vi "OPC Client.vi"(0 "Sequence Context In":refnum<k7>, 1 "Operations":T3(ring), 2 "Read":T2={"Value to Read"=enum."Flow Rate", "Timeout"=1.0}, 3 "Read Until":T1={"Timeout"=20.0, "Command"="FLOWRATE", "Measurement Interval"=1.0, "Lo Range Limit"=8.0, "Hi Range Limit"=4.0, "Delta Limit"=0.25, "Default Value"=0.0, "Value Done"=0.0, "Delta Value"=0.0, "Delta Time"=0.0}, 5 "error in":errorcluster, 8 "Comm":cluster{"Station":string, "Process name":string}={"Station"="OP30_1", "Process name"="RTheta"}, 9 "Time Out":cluster{"Continue Testing":bool, "Timeout":dbl}={"Continue Testing"=TRUE, "Timeout"=-1.0}) -> (13 "Fixture No.":string, 14 "comm ok?":bool, 15 "Code":string, 16 "Read Value":string, 17 "Read Until Value":dbl, 19 "error out":errorcluster)   [LabVIEW 2013]
uses:
  read_bool.vi
  read_String.vi
  <vilib>/addons/TestStand/_TSUtility.llb/TestStand - Get Property Value (Boolean).vi
  write_bool.vi
  read_Float.vi
  read_Num.vi
  write_Num.vi
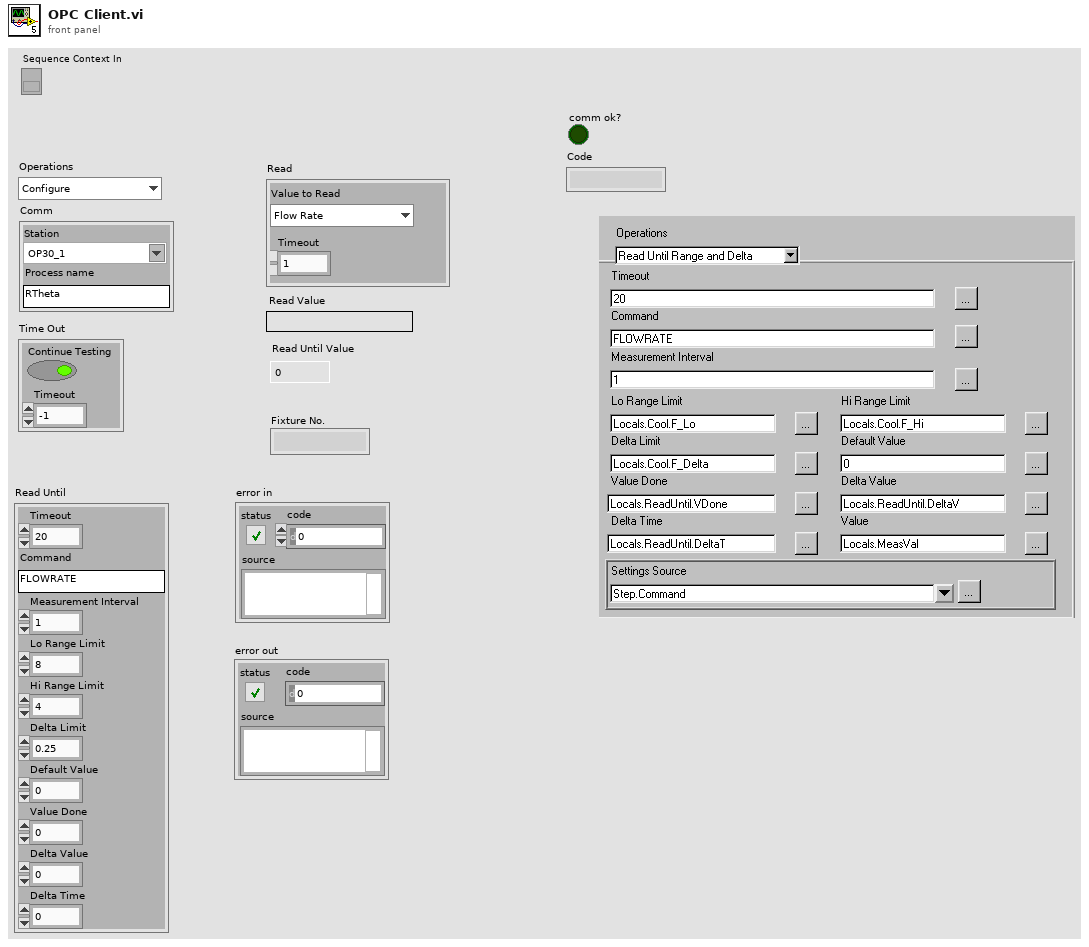
[diagram p1: front panel]
types:
  T1 = cluster{"Timeout":dbl, "Command":string, "Measurement Interval":dbl, "Lo Range Limit":dbl, "Hi Range Limit":dbl, "Delta Limit":dbl, "Default Value":dbl, "Value Done":dbl, "Delta Value":dbl, "Delta Time":dbl}
  T2 = cluster{"Value to Read":enum16{"Flow Rate", "Fluid Temp", "Fluid Fault State", "Temp Fault State", "Coolant Panel State", "Purge Complete", "Seal Test Complete", "Pressure"}, "Timeout":dbl}
  T3 = enum16{"Configure", "Process Name", "Wait Start Test", "Cool", "Read", "Read Until Range and Dellta", "Purge", "Pass", "Fail", "Retry", "Seal Test", "Close"}
  T4 = enum16{"Flow Rate", "Fluid Temp", "Fluid Fault State", "Temp Fault State", "Coolant Panel State", "Purge Complete", "Seal Test Complete", "Pressure"}
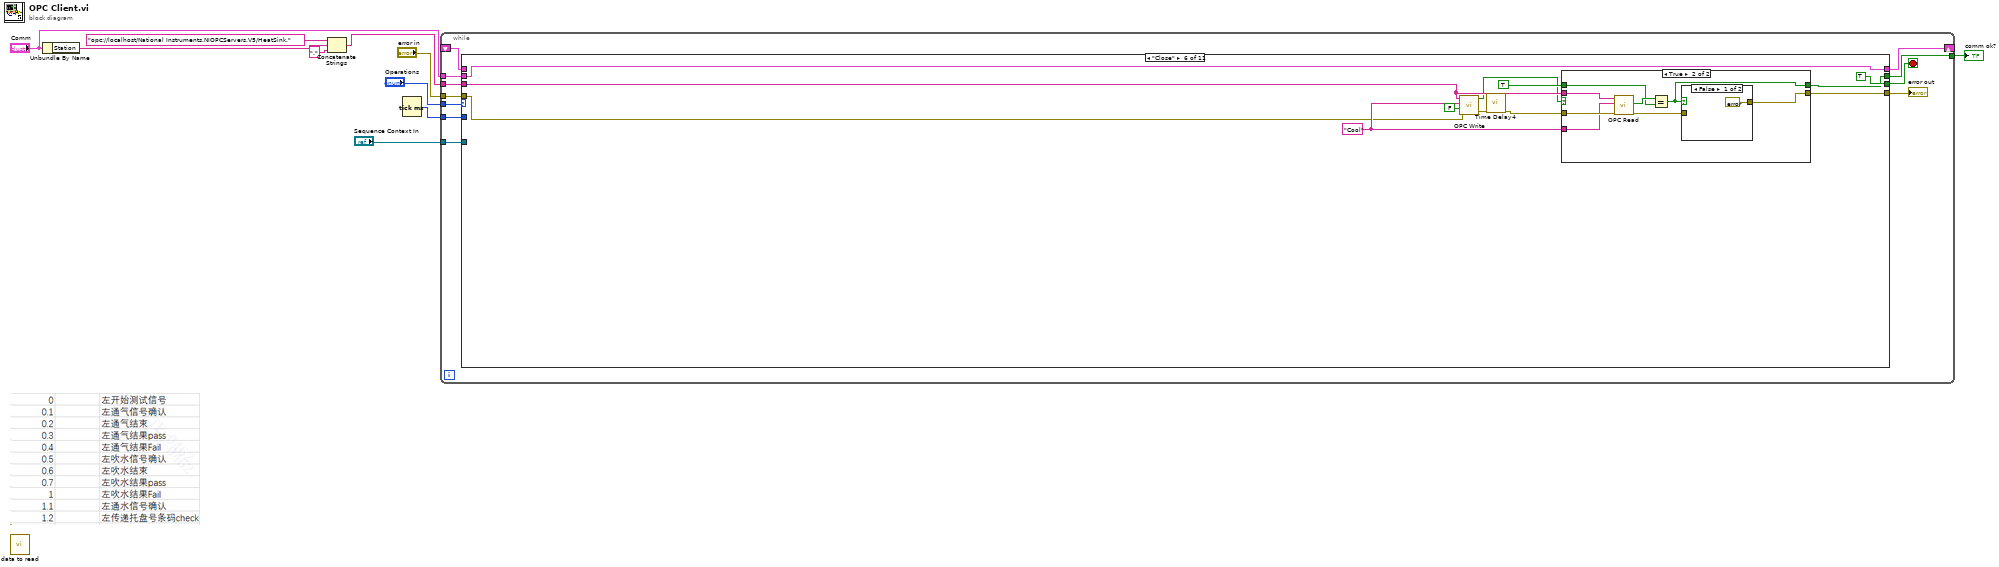
[diagram p0: block diagram]
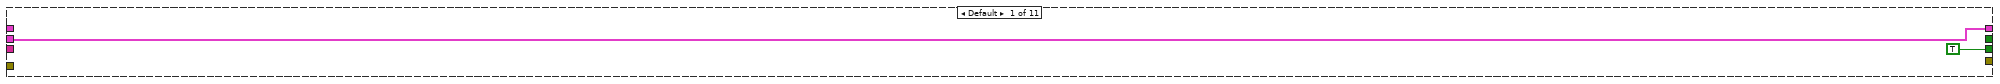
[diagram p2: hidden frame]
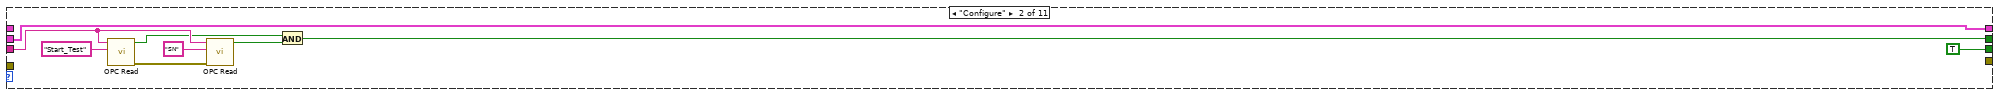
[diagram p3: hidden frame]
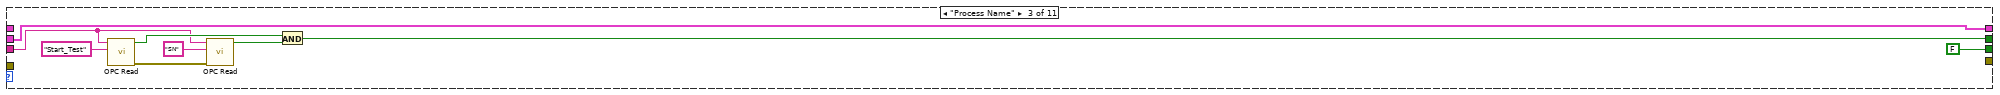
[diagram p4: hidden frame]
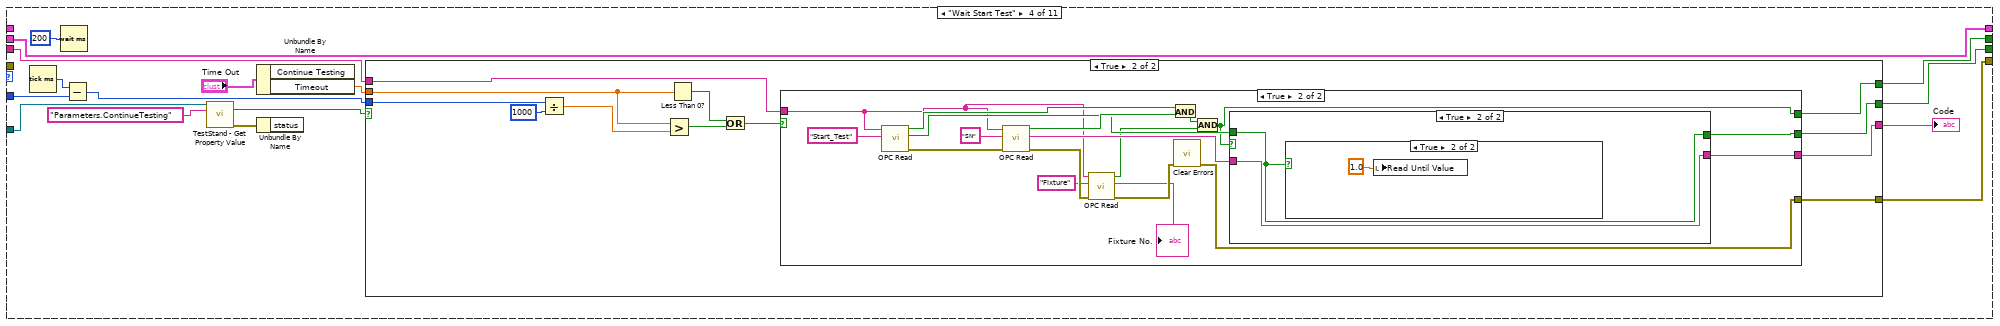
[diagram p5: hidden frame]
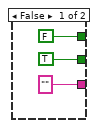
[diagram p6: hidden frame]
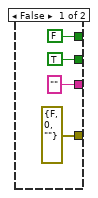
[diagram p7: hidden frame]
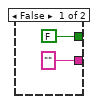
[diagram p8: hidden frame]
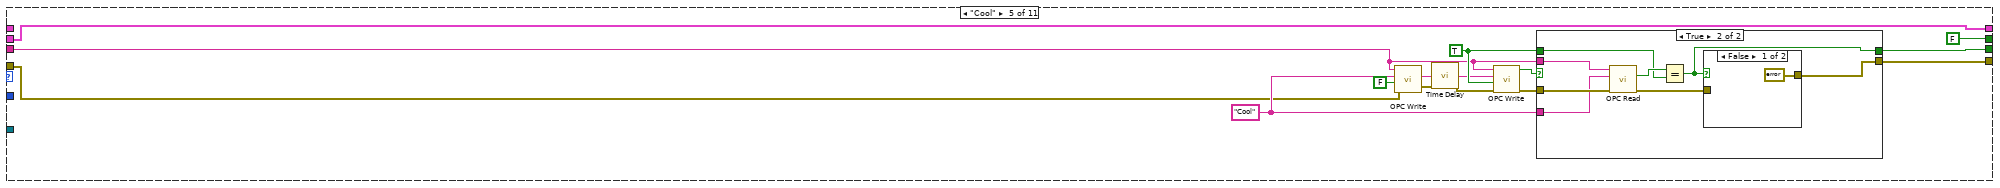
[diagram p10: hidden frame]
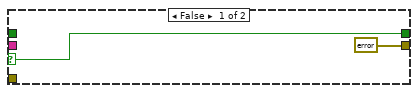
[diagram p11: hidden frame]
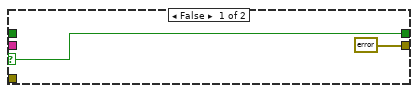
[diagram p13: hidden frame]
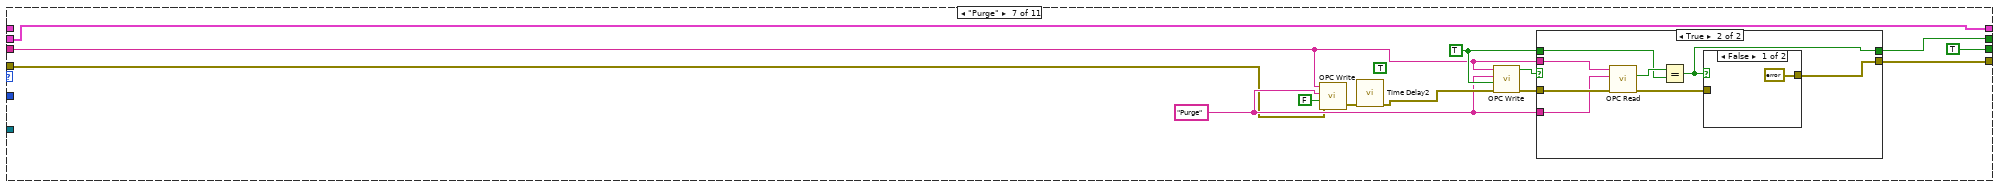
[diagram p15: hidden frame]
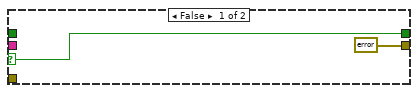
[diagram p16: hidden frame]
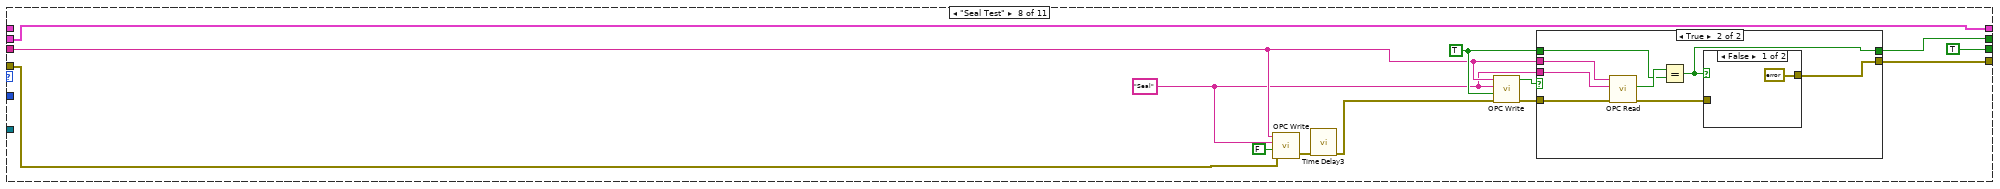
[diagram p18: hidden frame]
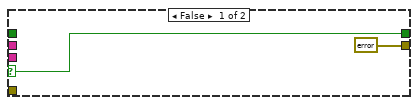
[diagram p19: hidden frame]
diagram:
  n1 = call "data to read.vi"() -> ()  [unwired: 9 in, 3 out]
  n2 = Unbundle By Name("Comm") -> ("Station"=w5:string)
  n3 = Concatenate Strings("opc://localhost/National Instruments.NIOPCServers.V5/HeatSink." ("URL"), w5, "." ("string")) -> (w8:string)
  n4 = Tick Count (ms)() -> (millisecond timer value=w3:u32)
  n5 = while {
    tunnel: w8 -> [w21]
    tunnel: "Operations" -> [w20]
    tunnel: "error in" -> [w19]
    shift-right: [w16] -> _
    shift-left: _ -> [w17]
    tunnel: "Comm" -> [w15]
    tunnel: w3 -> [w12]
    tunnel: "Sequence Context In" -> [w14]
    tunnel: [w11] -> w1
    stop <- w13 stop-if-true
    n6 = case shown="\"Close\"" w20 {
      selector: w20 -> [_ _ _ _ _ _ _ _ _ _ w421]
      tunnel: w21 -> [_ w28 w35 w55 w104 w132 w150 w176 w203 w350 w424]
      tunnel: [_ _ _ w54 w106 w134 w156 w184 w209 w341 w423] -> w18
      tunnel: w19 -> [_ _ _ _ w101 w129 w149 w177 w202 w342 w427]
      tunnel: w17 -> [_ _ _ _ _ _ _ _ _ _ _]
      tunnel: [w23 w32 w41 w57 w112 w136 w161 w183 w208 w353 w422] -> w16
      tunnel: w15 -> [w23 w32 w41 w57 w112 w136 w161 w183 w208 w353 w422]
      tunnel: w14 -> [_ _ _ w46 _ _ _ _ _ _ _]
      tunnel: [TRUE ("Value") TRUE ("Value") FALSE ("Value") w53 w107 TRUE TRUE ("Value") TRUE ("Value") TRUE ("Value") TRUE ("Value") TRUE ("Value")] -> w13
      tunnel: w12 -> [_ _ _ w49 _ _ _ _ _ _ _]
      tunnel: [_ w25 w34 w47 FALSE w125 w157 w181 w199 _ w418] -> w11
      frame Default {
      }
      frame "Configure" {
        n7 = call-poly "OPC Read.vi"("Address"="Start_Test", "URL"=w28) -> ("error out"=w29:errorcluster, "ok?"=w27:bool)  [unwired: 7 in, 1 out]
        n8 = call-poly "OPC Read.vi"("错误输入（无错误）"=w29, "Address"="SN", "URL"=w28) -> ("ok?"=w26:bool)  [unwired: 6 in, 2 out]
        n9 = And(x=w27, y=w26) -> (x .and. y?=w25:bool)
      }
      frame "Process Name" {
        n10 = call-poly "OPC Read.vi"("Address"="Start_Test", "URL"=w35) -> ("error out"=w38:errorcluster, "ok?"=w37:bool)  [unwired: 7 in, 1 out]
        n11 = call-poly "OPC Read.vi"("错误输入（无错误）"=w38, "Address"="SN", "URL"=w35) -> ("ok?"=w36:bool)  [unwired: 6 in, 2 out]
        n12 = And(x=w37, y=w36) -> (x .and. y?=w34:bool)
      }
      frame "Wait Start Test" {
        n13 = Tick Count (ms)() -> (millisecond timer value=w50:u32)
        n14 = Wait (ms)(milliseconds to wait=u32 200) -> ()  [unwired: 1 out]
        n15 = Subtract(x=w50, y=w49) -> (x-y=w48:u32)
        n16 = call-poly <vilib>:"TestStand - Get Property Value.vi"("Sequence Context In"=w46, "Lookup String"="Parameters.ContinueTesting") -> ("Value"=w44:bool, "error out"=w43:errorcluster)  [unwired: 11 in, 1 out]
        n17 = Unbundle By Name("Time Out") -> ("Timeout"=w51:dbl)  [unwired: 1 out]
        n18 = Unbundle By Name(w43) -> ()  [unwired: 1 out]
        n19 = case shown="True" w44 {
          tunnel: w55 -> [_ w72]
          tunnel: [_ w71] -> w54
          tunnel: [TRUE ("Value") w70] -> w53
          tunnel: ["" ("Value") w69] -> w52
          tunnel: w51 -> [_ w63]
          tunnel: w48 -> [_ w66]
          tunnel: [FALSE w61] -> w47
          frame False {
          }
          frame True {
            n20 = Divide(x=w66, y=u32 1000) -> (x/y=w64:dbl)
            n21 = Greater?(x=w63, y=w64) -> (0:w62:bool)
            n22 = Less Than 0?(x=w63) -> (x < 0?=w67:bool)
            n23 = Or(x=w67, y=w62) -> (x .or. y?=w68:bool)
            n24 = case shown="True" w68 {
              tunnel: w72 -> [_ w84]
              tunnel: [errorcluster {"status"=FALSE, "code"=0, "source"=""} ("error out") w91] -> w71
              tunnel: [TRUE ("Value") w87] -> w70
              tunnel: ["" ("Value") w85] -> w69
              tunnel: [FALSE w78] -> w61
              frame False {
              }
              frame True {
                n25 = call-poly "OPC Read.vi"("Address"="Start_Test", "URL"=w84) -> ("error out"=w92:errorcluster, "Value"=w88:bool, "ok?"=w90:bool)  [unwired: 7 in]
                n26 = call-poly "OPC Read.vi"("错误输入（无错误）"=w92, "Address"="SN", "URL"=w84) -> ("error out"=w83:errorcluster, "Value"=w86:string, "ok?"=w89:bool)  [unwired: 6 in]
                n27 = call-poly "OPC Read.vi"("错误输入（无错误）"=w83, "Address"="Fixture", "URL"=w84) -> ("error out"=w82:errorcluster, "Value"=→"Fixture No.":string, "ok?"=w79:bool)  [unwired: 6 in]
                n28 = And(x=w90, y=w89) -> (x .and. y?=w80:bool)
                n29 = call <vilib>:"Clear Errors.vi"("error in (no error)"=w82) -> ("error out"=w91:errorcluster)  [unwired: 6 in]
                n30 = And(x=w80, y=w79) -> (x .and. y?=w78:bool)
                n31 = case shown="True" w78 {
                  tunnel: w88 -> [_ w97]
                  tunnel: [FALSE ("Value") w97] -> w87
                  tunnel: w86 -> [_ w98]
                  tunnel: ["" ("Value") w98] -> w85
                  frame False {
                  }
                  frame True {
                    n32 = case shown="True" w97 {
                      frame False {
                      }
                      frame True {
                        n33 = local write "Read Until Value"(1.0 ("Read Until Value")) -> ()
                      }
                    }
                  }
                }
              }
            }
          }
        }
        "Code" <- w52
      }
      frame "Cool" {
        w108 = TRUE ("Value")
        w105 = "Cool" ("Address")
        n34 = call-poly "OPC Write.vi"("错误输入（无错误）"=w101, "Value"=FALSE, "Address"=w105, "URL"=w104) -> ("error out"=w102:errorcluster)  [unwired: 6 in, 1 out]
        n35 = call "Time Delay"("error in (no error)"=w102) -> ("error out"=w100:errorcluster)  [unwired: 10 in]
        n36 = call-poly "OPC Write.vi"("错误输入（无错误）"=w100, "Value"=w108, "Address"=w105, "URL"=w104) -> ("error out"=w109:errorcluster, "ok?"=w110:bool)  [unwired: 6 in]
        n37 = case shown="True" w110 {
          selector: w110 -> [w113 _]
          tunnel: w109 -> [_ w122]
          tunnel: w104 -> [_ w121]
          tunnel: [errorcluster {"status"=FALSE, "code"=10001, "source"="Write Error"} ("error out") w120] -> w106
          tunnel: [w113 w115] -> w107
          tunnel: w105 -> [_ w118]
          tunnel: w108 -> [_ w116]
          frame False {
          }
          frame True {
            n38 = call-poly "OPC Read.vi"("错误输入（无错误）"=w122, "Address"=w118, "URL"=w121) -> ("error out"=w119:errorcluster, "Value"=w117:bool)  [unwired: 6 in, 1 out]
            n39 = Equal?(x=w117, y=w116) -> (x = y?=w115:bool)
            n40 = case shown="False" w115 {
              tunnel: [errorcluster {"status"=FALSE, "code"=10001, "source"="Check Error"} ("error out") w124] -> w120
              tunnel: w119 -> [_ w124]
              frame False {
              }
              frame True {
              }
            }
          }
        }
      }
      frame "Close" {
        w133 = "Cool" ("Address")
        n41 = call-poly "OPC Write.vi"("错误输入（无错误）"=w129, "Value"=FALSE, "Address"=w133, "URL"=w132) -> ("error out"=w130:errorcluster, "ok?"=w127:bool)  [unwired: 6 in]
        n42 = call "Time Delay4"("error in (no error)"=w130) -> ("error out"=w128:errorcluster)  [unwired: 10 in]
        n43 = case shown="True" w127 {
          selector: w127 -> [w137 _]
          tunnel: w128 -> [_ w146]
          tunnel: w132 -> [_ w145]
          tunnel: [errorcluster {"status"=FALSE, "code"=10001, "source"="Write Error"} ("error out") w144] -> w134
          tunnel: [w137 w139] -> w125
          tunnel: w133 -> [_ w142]
          tunnel: TRUE ("Value") -> [_ w140]
          frame False {
          }
          frame True {
            n44 = call-poly "OPC Read.vi"("错误输入（无错误）"=w146, "Address"=w142, "URL"=w145) -> ("error out"=w143:errorcluster, "Value"=w141:bool)  [unwired: 6 in, 1 out]
            n45 = Equal?(x=w141, y=w140) -> (x = y?=w139:bool)
            n46 = case shown="False" w139 {
              tunnel: [errorcluster {"status"=FALSE, "code"=10001, "source"="Check Error"} ("error out") w148] -> w144
              tunnel: w143 -> [_ w148]
              frame False {
              }
              frame True {
              }
            }
          }
        }
      }
      frame "Purge" {
        (unwired) TRUE ("Value")
        w158 = TRUE ("Value")
        w151 = "Purge" ("Address")
        n47 = call-poly "OPC Write.vi"("错误输入（无错误）"=w149, "Value"=FALSE, "Address"=w151, "URL"=w150) -> ("error out"=w153:errorcluster)  [unwired: 6 in, 1 out]
        n48 = call "Time Delay2"("error in (no error)"=w153) -> ("error out"=w152:errorcluster)  [unwired: 10 in]
        n49 = call-poly "OPC Write.vi"("错误输入（无错误）"=w152, "Value"=w158, "Address"=w151, "URL"=w150) -> ("error out"=w159:errorcluster, "ok?"=w160:bool)  [unwired: 6 in]
        n50 = case shown="True" w160 {
          selector: w160 -> [w162 _]
          tunnel: w159 -> [_ w171]
          tunnel: w150 -> [_ w170]
          tunnel: [errorcluster {"status"=FALSE, "code"=10001, "source"="Write Error"} ("error out") w169] -> w156
          tunnel: [w162 w164] -> w157
          tunnel: w151 -> [_ w167]
          tunnel: w158 -> [_ w165]
          frame False {
          }
          frame True {
            n51 = call-poly "OPC Read.vi"("错误输入（无错误）"=w171, "Address"=w167, "URL"=w170) -> ("error out"=w168:errorcluster, "Value"=w166:bool)  [unwired: 6 in, 1 out]
            n52 = Equal?(x=w166, y=w165) -> (x = y?=w164:bool)
            n53 = case shown="False" w164 {
              tunnel: [errorcluster {"status"=FALSE, "code"=10001, "source"="Check Error"} ("error out") w173] -> w169
              tunnel: w168 -> [_ w173]
              frame False {
              }
              frame True {
              }
            }
          }
        }
      }
      frame "Seal Test" {
        w182 = TRUE ("Value")
        w175 = "Seal" ("Address")
        n54 = call-poly "OPC Write.vi"("错误输入（无错误）"=w177, "Value"=FALSE, "Address"=w175, "URL"=w176) -> ("error out"=w178:errorcluster)  [unwired: 6 in, 1 out]
        n55 = call "Time Delay3"("error in (no error)"=w178) -> ("error out"=w174:errorcluster)  [unwired: 10 in]
        n56 = call-poly "OPC Write.vi"("错误输入（无错误）"=w174, "Value"=w182, "Address"=w175, "URL"=w176) -> ("error out"=w185:errorcluster, "ok?"=w186:bool)  [unwired: 6 in]
        n57 = case shown="True" w186 {
          selector: w186 -> [w187 _]
          tunnel: w185 -> [_ w196]
          tunnel: w176 -> [_ w195]
          tunnel: [errorcluster {"status"=FALSE, "code"=10001, "source"="Write Error"} ("error out") w194] -> w184
          tunnel: [w187 w189] -> w181
          tunnel: w175 -> [_ w192]
          tunnel: w182 -> [_ w190]
          frame False {
          }
          frame True {
            n58 = call-poly "OPC Read.vi"("错误输入（无错误）"=w196, "Address"=w192, "URL"=w195) -> ("error out"=w193:errorcluster, "Value"=w191:bool)  [unwired: 6 in, 1 out]
            n59 = Equal?(x=w191, y=w190) -> (x = y?=w189:bool)
            n60 = case shown="False" w189 {
              tunnel: [errorcluster {"status"=FALSE, "code"=10001, "source"="Check Error"} ("error out") w198] -> w194
              tunnel: w193 -> [_ w198]
              frame False {
              }
              frame True {
              }
            }
          }
        }
      }
      frame "Read" {
        # "1.3-1.6      Seal Cool Purge Bypass\n\n4.3-4.6      Seal Cool Purge Bypass"
        n61 = Unbundle By Name("Read") -> ("Value to Read"=w205:T4)  [unwired: 1 out]
        n62 = case shown="\"Temp Fault State\"" w205 {
          tunnel: ["None" ("Read Value") w215 w225 w242 w269 w281 w299 w312 w331] -> w204
          tunnel: w203 -> [_ w220 w223 w235 w260 w285 w298 w315 w332]
          tunnel: w202 -> [w211 w219 w226 w247 w268 w284 w297 w314 w329]
          tunnel: [w211 w218 w222 w239 w261 w283 w296 w313 w328] -> w201
          tunnel: [TRUE ("ok?") w213 w221 w236 w258 w279 w295 w311 w327] -> w199
          frame Default {
          }
          frame "Flow Rate" {
            n63 = call-poly "OPC Read.vi"("错误输入（无错误）"=w219, "Address"="FlowRate", "URL"=w220) -> ("error out"=w218:errorcluster, "Value"=w214:dbl, "ok?"=w213:bool)  [unwired: 6 in]
            n64 = local write "Read Until Value"(w214) -> ()
            n65 = Format Into String(initial string="%.3f", w214) -> (resulting string=w215:string)  [unwired: 2 in, 1 out]
          }
          frame "Fluid Temp" {
            n66 = call-poly "OPC Read.vi"("错误输入（无错误）"=w226, "Address"="FluidTemp", "URL"=w223) -> ("error out"=w222:errorcluster, "Value"=w224:dbl, "ok?"=w221:bool)  [unwired: 6 in]
            n67 = local write "Read Until Value"(w224) -> ()
            n68 = Format Into String(initial string="%.3f", w224) -> (resulting string=w225:string)  [unwired: 2 in, 1 out]
          }
          frame "Fluid Fault State" {
            n69 = call-poly "OPC Read.vi"("错误输入（无错误）"=w247, "Address"="CoolantState", "URL"=w235) -> ("error out"=w240:errorcluster, "Value"=w246:i32, "ok?"=w237:bool)  [unwired: 6 in]
            n70 = Number To Boolean Array(number=w246) -> (Boolean array=w245:bool[])
            n71 = call-poly "OPC Read.vi"("错误输入（无错误）"=w240, "Address"="FlowRate", "URL"=w235) -> ("error out"=w239:errorcluster, "Value"=w234:dbl, "ok?"=w238:bool)  [unwired: 6 in]
            n72 = for {
              tunnel: w245 -> [w253]
              tunnel: [w252] -> w243 mode=indexing
              tunnel: i32[] [4] -> [w251] mode=indexing
              n73 = Index Array(array=w253, index=w251) -> (element=w252:bool)
            }
            n74 = And(x=w237, y=w238) -> (x .and. y?=w236:bool)
            n75 = In Range and Coerce(upper limit=12.0, x=w234, lower limit=4.0) -> (In Range?=w231:bool)  [unwired: 1 out]
            n76 = And Array Elements(Boolean array=w243) -> (logical AND=w230:bool)
            n77 = And(x=w230, y=w231) -> (x .and. y?=w229:bool)
            n78 = case shown="False" w229 {
              tunnel: ["FLOW OUT TOLERANCE" ("Read Value") "FLOW IN TOLERANCE" ("Read Value")] -> w242
              frame False {
              }
              frame True {
              }
            }
          }
          frame "Temp Fault State" {
            n79 = call-poly "OPC Read.vi"("错误输入（无错误）"=w268, "Address"="CoolantState", "URL"=w260) -> ("error out"=w262:errorcluster, "Value"=w272:i32, "ok?"=w259:bool)  [unwired: 6 in]
            n80 = call-poly "OPC Read.vi"("错误输入（无错误）"=w262, "Address"="FluidTemp", "URL"=w260) -> ("error out"=w261:errorcluster, "Value"=w265:dbl, "ok?"=w256:bool)  [unwired: 6 in]
            n81 = Number To Boolean Array(number=w272) -> (Boolean array=w271:bool[])
            n82 = In Range and Coerce(upper limit=80.0, x=w265, lower limit=50.0) -> (In Range?=w254:bool)  [unwired: 1 out]
            n83 = for {
              tunnel: w271 -> [w278]
              tunnel: [w277] -> w270 mode=indexing
              tunnel: i32[] [4] -> [w276] mode=indexing
              n84 = Index Array(array=w278, index=w276) -> (element=w277:bool)
            }
            n85 = And(x=w259, y=w256) -> (x .and. y?=w258:bool)
            n86 = And Array Elements(Boolean array=w270) -> (logical AND=w257:bool)
            n87 = And(x=w257, y=w254) -> (x .and. y?=w255:bool)
            n88 = case shown="False" w255 {
              tunnel: ["TEMP OUT TOLERANCE" ("Read Value") "TEMP IN TOLERANCE" ("Read Value")] -> w269
              frame False {
              }
              frame True {
              }
            }
          }
          frame "Coolant Panel State" {
            n89 = call-poly "OPC Read.vi"("错误输入（无错误）"=w284, "Address"="CoolantState", "URL"=w285) -> ("error out"=w283:errorcluster, "Value"=w288:i32, "ok?"=w279:bool)  [unwired: 6 in]
            n90 = Number To Boolean Array(number=w288) -> (Boolean array=w287:bool[])
            n91 = for {
              tunnel: w287 -> [w294]
              tunnel: [w293] -> w282 mode=indexing
              tunnel: i32[] [3, 4, 5, 6] -> [w292] mode=indexing
              n92 = Index Array(array=w294, index=w292) -> (element=w293:bool)
            }
            n93 = for {
              tunnel: w282 -> [w290] mode=indexing
              tunnel: [w291] -> w281
              tunnel: string[] ["SEAL", "COOL", "PURGE", "BYPASSED"] -> [w291] mode=indexing
              stop <- w290 stop-if-true
            }
          }
          frame "Purge Complete" {
            n94 = call-poly "OPC Read.vi"("错误输入（无错误）"=w297, "Address"="CoolantResult", "URL"=w298) -> ("error out"=w296:errorcluster, "Value"=w304:i32, "ok?"=w295:bool)  [unwired: 6 in]
            n95 = Number To Boolean Array(number=w304) -> (Boolean array=w303:bool[])
            n96 = for {
              tunnel: w303 -> [w310]
              tunnel: [w309] -> w301 mode=indexing
              tunnel: i32[] [6, 7] -> [w308] mode=indexing
              n97 = Index Array(array=w310, index=w308) -> (element=w309:bool)
            }
            n98 = And Array Elements(Boolean array=w301) -> (logical AND=w300:bool)
            n99 = case shown="False" w300 {
              tunnel: ["PURGE NG......" ("Read Value") "PURGECOMPLETE" ("Read Value")] -> w299
              frame False {
              }
              frame True {
              }
            }
          }
          frame "Seal Test Complete" {
            n100 = call-poly "OPC Read.vi"("错误输入（无错误）"=w314, "Address"="CoolantResult", "URL"=w315) -> ("error out"=w313:errorcluster, "Value"=w320:i32, "ok?"=w311:bool)  [unwired: 6 in]
            n101 = Number To Boolean Array(number=w320) -> (Boolean array=w319:bool[])
            n102 = for {
              tunnel: w319 -> [w326]
              tunnel: [w325] -> w317 mode=indexing
              tunnel: i32[] [2, 3] -> [w324] mode=indexing
              n103 = Index Array(array=w326, index=w324) -> (element=w325:bool)
            }
            n104 = And Array Elements(Boolean array=w317) -> (logical AND=w316:bool)
            n105 = case shown="False" w316 {
              tunnel: ["ST NG......" ("Read Value") "STCOMPLETE......" ("Read Value")] -> w312
              frame False {
              }
              frame True {
              }
            }
          }
          frame "Pressure" {
            n106 = call-poly "OPC Read.vi"("错误输入（无错误）"=w329, "Address"="Pressure", "URL"=w332) -> ("error out"=w328:errorcluster, "Value"=w330:dbl, "ok?"=w327:bool)  [unwired: 6 in]
            n107 = local write "Read Until Value"(w330) -> ()
            n108 = Format Into String(initial string="%.3f", w330) -> (resulting string=w331:string)  [unwired: 2 in, 1 out]
          }
        }
        n109 = case shown="True" w199 {
          tunnel: [errorcluster {"status"=FALSE, "code"=10001, "source"="Check Error"} ("error out") w338] -> w209
          tunnel: w201 -> [_ w338]
          tunnel: ["Timeout" ("Read Value") w337] -> w206
          tunnel: w204 -> [_ w337]
          frame False {
          }
          frame True {
          }
        }
        "Read Value" <- w206
      }
      frame "Read Until Range and Dellta" {
        n110 = Unbundle By Name("Read Until") -> ("Timeout"=w348:dbl, "Command"=w351:string, "Measurement Interval"=w347:dbl, "Lo Range Limit"=w343:dbl, "Hi Range Limit"=w344:dbl, "Delta Limit"=w340:dbl)  [unwired: 2 out]
        n111 = Tick Count (ms)() -> (millisecond timer value=w349:u32)
        n112 = while {
          tunnel: w351 -> [w375]
          tunnel: w350 -> [w374]
          tunnel: w349 -> [w354]
          tunnel: w348 -> [w369]
          tunnel: w347 -> [w367]
          shift-right: [w365] -> w345
          shift-left: 0.0 ("Value") -> [w361]
          tunnel: w344 -> [w360]
          tunnel: w343 -> [w359]
          tunnel: w342 -> [w358]
          tunnel: [w357] -> w341
          tunnel: w340 -> [w356]
          stop <- w368 stop-if-true
          n113 = Wait (ms)(milliseconds to wait=u32 20) -> ()  [unwired: 1 out]
          n114 = call "Elapsed Time"("Time Target (s)"=w367, "Auto Reset"=TRUE) -> ("Time has Elapsed"=w364:bool)  [unwired: 10 in, 7 out]
          n115 = case shown="True" w364 {
            tunnel: w375 -> [_ w395]
            tunnel: w374 -> [_ w394]
            tunnel: [w376 w391] -> w365
            tunnel: [FALSE ("ok?") w387] -> w362
            tunnel: w361 -> [w376 w392]
            tunnel: w360 -> [_ w390]
            tunnel: w359 -> [_ w389]
            tunnel: w358 -> [w377 w386]
            tunnel: [w377 w385] -> w357
            tunnel: w356 -> [_ w382]
            frame False {
            }
            frame True {
              n116 = case shown="\"FLOWRATE\"" w395 {
                tunnel: w394 -> [w401 w407 w413 _]
                tunnel: [w399 w405 w411 0.0 ("Value")] -> w391
                tunnel: [w396 w402 w410 TRUE ("ok?")] -> w393
                tunnel: w386 -> [w398 w404 w409 w415]
                tunnel: [w397 w403 w408 w415] -> w385
                frame "FLOWRATE" {
                  n117 = call-poly "OPC Read.vi"("错误输入（无错误）"=w398, "Address"="FlowRate", "URL"=w401) -> ("error out"=w397:errorcluster, "Value"=w399:dbl, "ok?"=w396:bool)  [unwired: 6 in]
                }
                frame "FLUIDTEMP" {
                  n118 = call-poly "OPC Read.vi"("错误输入（无错误）"=w404, "Address"="FluidTemp", "URL"=w407) -> ("error out"=w403:errorcluster, "Value"=w405:dbl, "ok?"=w402:bool)  [unwired: 6 in]
                }
                frame "PRESSURE" {
                  n119 = call-poly "OPC Read.vi"("错误输入（无错误）"=w409, "Address"="Pressure", "URL"=w413) -> ("error out"=w408:errorcluster, "Value"=w411:dbl, "ok?"=w410:bool)  [unwired: 6 in]
                }
                frame Default {
                }
              }
              n120 = In Range and Coerce(upper limit=w390, x=w391, lower limit=w389) -> (In Range?=w381:bool)  [unwired: 1 out]
              n121 = Subtract(x=w391, y=w392) -> (x-y=w384:dbl)
              n122 = Absolute Value(x=w384) -> (abs(x)=w383:dbl)
              n123 = Less Or Equal?(x=w383, y=w382) -> (x <= y?=w380:bool)
              n124 = And(x=w381, y=w380) -> (x .and. y?=w379:bool)
              n125 = Not(x=w393) -> (.not. x?=w388:bool)
              n126 = Or(x=w388, y=w379) -> (x .or. y?=w387:bool)
            }
          }
          n127 = Tick Count (ms)() -> (millisecond timer value=w355:u32)
          n128 = Subtract(x=w355, y=w354) -> (x-y=w373:u32)
          n129 = Divide(x=w373, y=u32 1000) -> (x/y=w370:dbl)
          n130 = Greater Or Equal?(x=w370, y=w369) -> (x >= y?=w363:bool)
          n131 = Or(x=w362, y=w363) -> (x .or. y?=w368:bool)
        }
        "Read Until Value" <- w345
      }
      frame "Pass".."Retry" {
        w419 = "Result" ("Address")
        # "0.0\tfis end\n0.1\tend\n0.2\tpass\n0.3 \tfail\n0.4\tFis Pass\n0.5\tFIS Fail\n0.6\tIntest\n0.7\tRetry\n\n1618\n0.0\tfis end\n0.1\tend\n0.2\tpass\n0.3 \tfail\n0.4\tFis Pass\n0.5\tFIS Fail\n0.6\tIntest\n0.7\tRetry"
        n132 = case shown="\"Fail\"" w421 {
          tunnel: [0 ("Value") 6 ("Value") 10 ("Value") 130 ("Value")] -> w420
          frame Default {
          }
          frame "Pass" {
          }
          frame "Fail" {
          }
          frame "Retry" {
          }
        }
        n133 = call-poly "OPC Write.vi"("错误输入（无错误）"=w427, "Value"=w420, "Address"=w419, "URL"=w424) -> ("error out"=w425:errorcluster, "ok?"=w426:bool)  [unwired: 6 in]
        n134 = case shown="True" w426 {
          selector: w426 -> [w432 _]
          tunnel: w425 -> [_ w443]
          tunnel: w424 -> [_ w442]
          tunnel: [errorcluster {"status"=FALSE, "code"=10001, "source"="Write Error"} ("error out") w437] -> w423
          tunnel: w420 -> [_ w441]
          tunnel: [w432 w438] -> w418
          tunnel: w419 -> [_ w435]
          frame False {
          }
          frame True {
            n135 = call-poly "OPC Read.vi"("错误输入（无错误）"=w443, "Address"=w435, "URL"=w442) -> ("error out"=w436:errorcluster, "Value"=w434:i32, "ok?"=w439:bool)  [unwired: 6 in]
            n136 = Equal?(x=w441, y=w434) -> (x = y?=w440:bool)
            n137 = And(x=w439, y=w440) -> (x .and. y?=w438:bool)
            n138 = case shown="False" w438 {
              tunnel: [errorcluster {"status"=FALSE, "code"=10001, "source"="Check Error"} ("error out") w445] -> w437
              tunnel: w436 -> [_ w445]
              frame False {
              }
              frame True {
              }
            }
          }
        }
      }
    }
    "error out" <- w18
  }
  "comm ok?" <- w1
